vi "Read Configuration.vi"(8 "error in (no error)":errorcluster, 11 "Process In":refnum<class "Process.lvclass">) -> (0 "error out":errorcluster, 3 "Process Out":refnum<class "Process.lvclass">)   [LabVIEW 2020, in "Process.lvclass"]
doc: "Sub-classes may override this VI, which should read default configurations from the configuration source or potentially configure hard coded values. This VI is called from within the process loop the first time the process is started using the Start.vi.\nIt is important to set the configured attributes by value and not send commands to the process loop as there might be other messages in the queue which which will then be handled before the loading of the configuration is completed."
uses:
  Process.lvclass
  Process.lvclass/Process.ctl
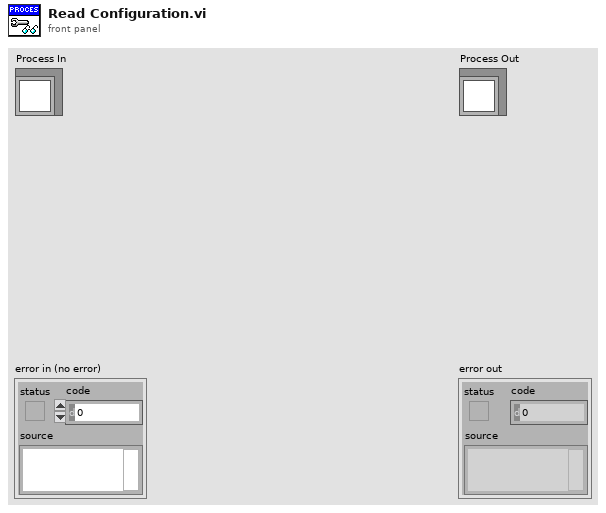
[diagram p1: front panel]
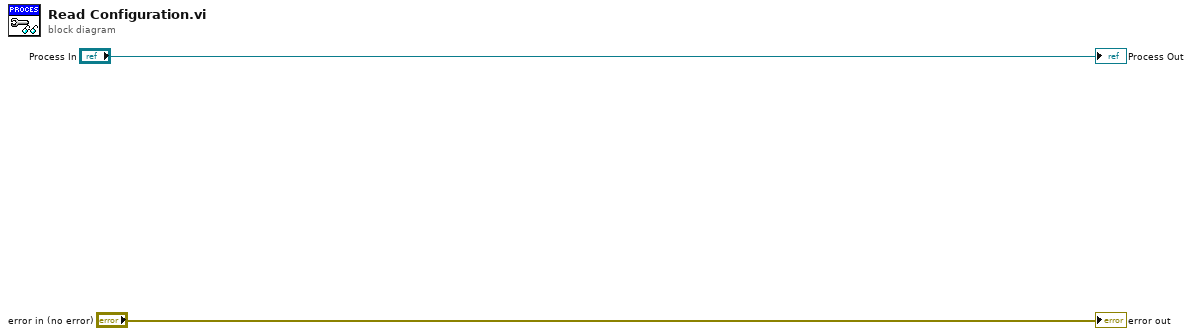
[diagram p0: block diagram]
diagram:
  "error out" <- "error in (no error)"
  "Process Out" <- "Process In"
